vi "Write OPC UA Ref.vi"(8 "error in (no error)":errorcluster, 10 "OPC UA client refnum":T1, 11 "Abstract in":refnum<class "Abstract.lvclass">) -> (0 "error out":errorcluster, 3 "Abstract out":refnum<class "Abstract.lvclass">)   [LabVIEW 2025, in "Abstract.lvclass"]
uses:
  Abstract.lvclass
  <vilib>/OPCUA/controls/OPC UA Client Refnum.ctl
  Abstract.lvclass/Abstract.ctl
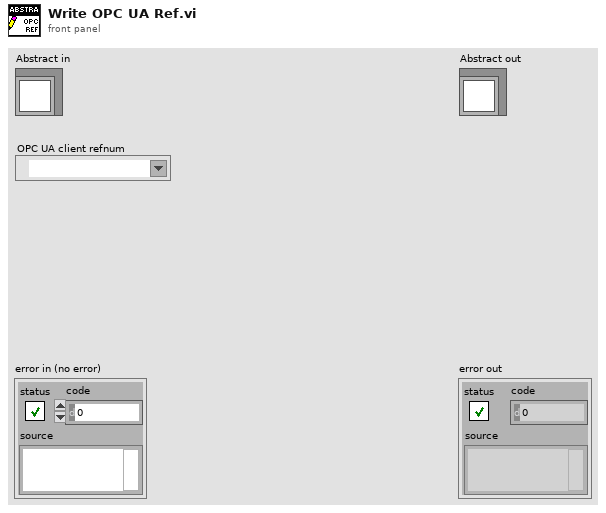
[diagram p1: front panel]
types:
  T1 = typedef "OPC UA Client Refnum.ctl" = refnum<k21>
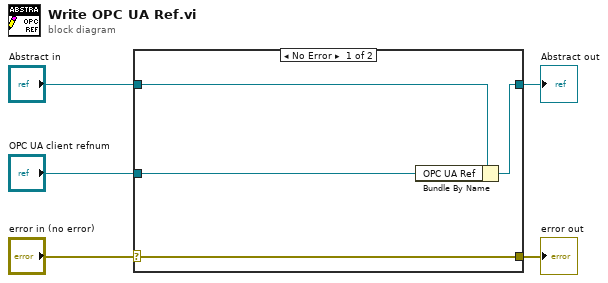
[diagram p0: block diagram]
diagram:
  n1 = case shown="No Error" "error in (no error)" {
    selector: "error in (no error)" -> [w9 w10]
    tunnel: [w9 w10] -> w4
    tunnel: [w7 w11] -> w2
    tunnel: "Abstract in" -> [w8 w11]
    tunnel: "OPC UA client refnum" -> [w6 _]
    frame No Error {
      n2 = Bundle By Name(cluster=w8, "OPC UA Ref"=w6) -> (w7:refnum<class "Abstract.lvclass">)
    }
    frame Error {
    }
  }
  "error out" <- w4
  "Abstract out" <- w2
